vi "MouseDown.vi"(7 "Flip colors?":bool, 8 "error in":errorcluster, 10 "Coords":T5, 11 "Data in":T1={"Class"={"Ants"=refnum, "Layer"=refnum, "Templates"=refnum, "Icon"=refnum, "Glyph"=refnum, "Settings"=refnum, "Tools"=refnum, "History"=refnum}, "Ref"={"Add Layer"=refnum, "Remove Layer"=refnum, "Line Text"=[], "Body Text Spec"=refnum, "DNL_Font"=refnum, "glyph path str"=refnum, "templates path str"=refnum, "Arrow Up"=refnum, "Arrow Down"=refnum, "IE VI Ref"=refnum, "Glyphs tree"=refnum, "Templates tree"=refnum, "Layer Icon Text"=refnum, "Layer Template"=refnum, "Body Text"=refnum, "Search Templates"=refnum, "TextMarker"=refnum, "Tab Control"=refnum, "Search Glyphs"=refnum, "Line Color"=refnum, "DNL_Glyphs []"=refnum, "Fill Color"=refnum, "Tools"=refnum, "Icon"=refnum, "Preview"=refnum, "Ants"=refnum, "Terminals"=refnum, "menu reference"=refnum, "LayerNames"=[], "GlyphLoadAnimation"=refnum, "TemplateLoadAnimation"=refnum, "refreshGlyphs"=refnum, "refreshTemplates"=refnum}, "Support"={"AntsRect"={"left"=0, "top"=0, "right"=0, "bottom"=0}, "Mouse Move Coords"={"Horizontal"=0, "Vertical"=0}, "Mouse Down Coords"={"Horizontal"=0, "Vertical"=0}, "Temp Coord"={"Horizontal"=0, "Vertical"=0}, "Action"=enum."Default", "Edge Color"=4914962, "Fill Color"=16860, "Mouse Down?"=FALSE, "Draft Mode?"=FALSE, "Temp Icon"=bytes[3102], "CTRL Pressed"=FALSE, "Move Selection?"=FALSE, "AntsRect Orig"={"left"=0, "top"=0, "right"=0, "bottom"=0}, "Text"="", "TM Set?"=FALSE, "Mouse inside icon?"=FALSE, "Tool (old value)"=0, "Pencil Move Color"=0, "Swap Colors?"=FALSE, "Shift pressed?"=FALSE}}) -> (0 "error out":errorcluster, 3 "Data out":T1={"Class"={"Ants"=refnum, "Layer"=refnum, "Templates"=refnum, "Icon"=refnum, "Glyph"=refnum, "Settings"=refnum, "Tools"=refnum, "History"=refnum}, "Ref"={"Add Layer"=refnum, "Remove Layer"=refnum, "Line Text"=[], "Body Text Spec"=refnum, "DNL_Font"=refnum, "glyph path str"=refnum, "templates path str"=refnum, "Arrow Up"=refnum, "Arrow Down"=refnum, "IE VI Ref"=refnum, "Glyphs tree"=refnum, "Templates tree"=refnum, "Layer Icon Text"=refnum, "Layer Template"=refnum, "Body Text"=refnum, "Search Templates"=refnum, "TextMarker"=refnum, "Tab Control"=refnum, "Search Glyphs"=refnum, "Line Color"=refnum, "DNL_Glyphs []"=refnum, "Fill Color"=refnum, "Tools"=refnum, "Icon"=refnum, "Preview"=refnum, "Ants"=refnum, "Terminals"=refnum, "menu reference"=refnum, "LayerNames"=[], "GlyphLoadAnimation"=refnum, "TemplateLoadAnimation"=refnum, "refreshGlyphs"=refnum, "refreshTemplates"=refnum}, "Support"={"AntsRect"={"left"=0, "top"=0, "right"=0, "bottom"=0}, "Mouse Move Coords"={"Horizontal"=0, "Vertical"=0}, "Mouse Down Coords"={"Horizontal"=0, "Vertical"=0}, "Temp Coord"={"Horizontal"=0, "Vertical"=0}, "Action"=enum."Default", "Edge Color"=4914962, "Fill Color"=16860, "Mouse Down?"=FALSE, "Draft Mode?"=FALSE, "Temp Icon"=bytes[3102], "CTRL Pressed"=FALSE, "Move Selection?"=FALSE, "AntsRect Orig"={"left"=0, "top"=0, "right"=0, "bottom"=0}, "Text"="", "TM Set?"=FALSE, "Mouse inside icon?"=FALSE, "Tool (old value)"=0, "Pencil Move Color"=0, "Swap Colors?"=FALSE, "Shift pressed?"=FALSE}})   [LabVIEW 2020]
uses:
  Class/Ants/Ants.lvclass
  Class/FakedArray/FakedArray.lvclass
  vi.lib/LabVIEW Icon API/lv_icon/Classes/Icon/Icon.lvclass
  Class/Icon Library/Glyph.lvclass
  Class/Settings/Settings.lvclass
  Class/Tools/Tools Paint.lvclass
  History/History/History.lvclass
  Controls/SupportClass_Action.ctl
  History/History.lvlib
  <vilib>/Utility/miscctls.llb/LVPoint32TypeDef.ctl
  vi.lib/LabVIEW Icon API/lv_icon/Controls/IEColor.ctl
  Controls/Support Cluster.ctl
  lv_icon.lvlib
  Controls/References Cluster.ctl
  Controls/IE Classes.ctl
  Controls/Global Data.ctl
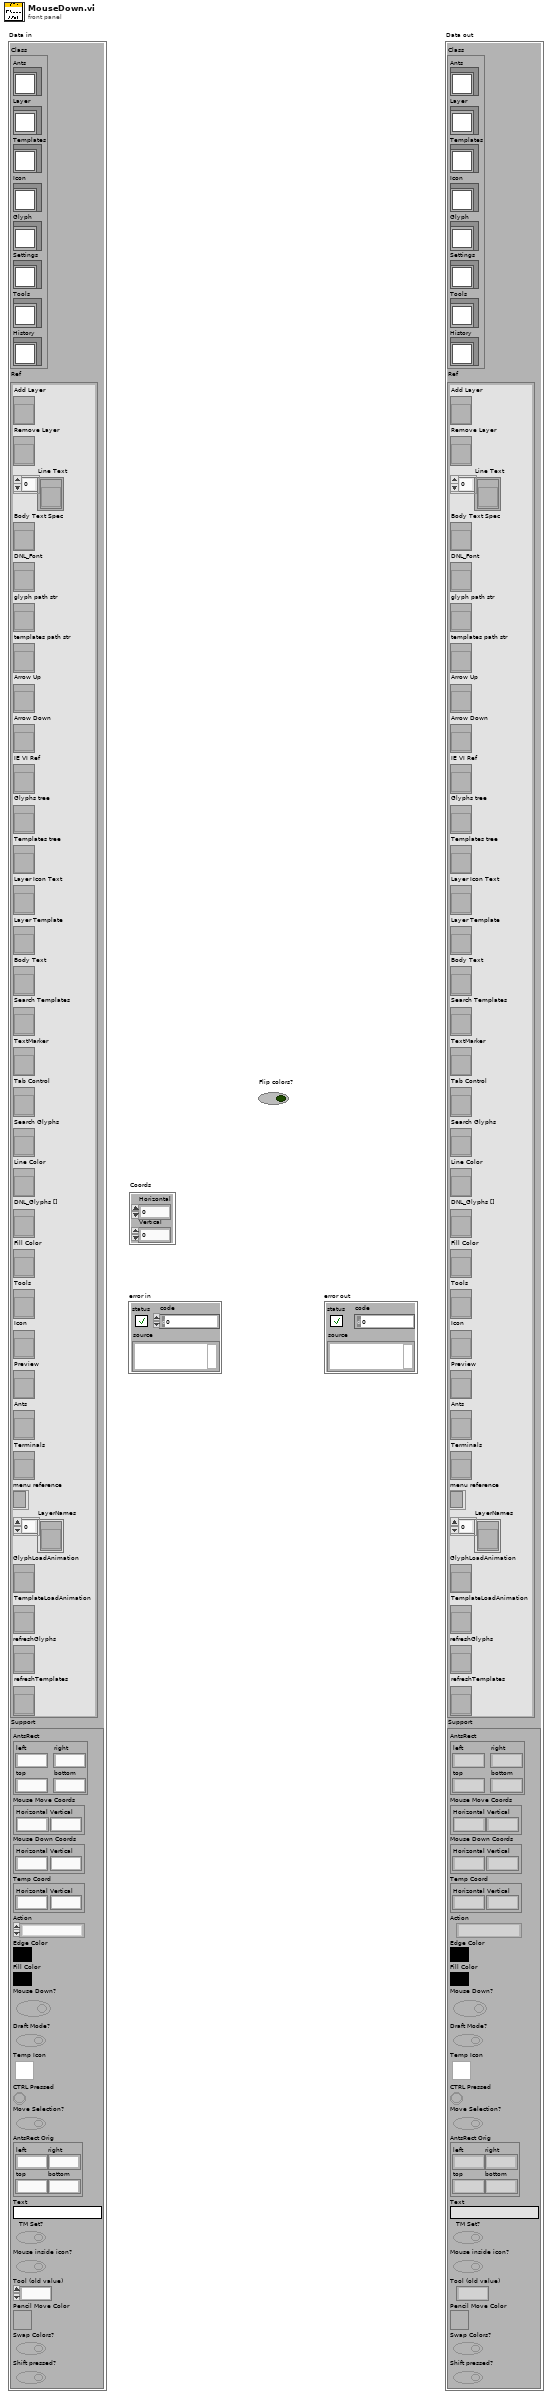
[diagram p1: front panel]
types:
  T1 = typedef "lv_icon.lvlib/Global Data.ctl" = cluster{"Class":T2, "Ref":T3, "Support":T4}
  T2 = typedef "lv_icon.lvlib/IE Classes.ctl" = cluster{"Ants":refnum<class "Ants.lvclass">, "Layer":refnum<class "FakedArray.lvclass">, "Templates":refnum<class "FakedArray.lvclass">, "Icon":refnum<class "Icon.lvclass">, "Glyph":refnum<class "Glyph.lvclass">, "Settings":refnum<class "Settings.lvclass">, "Tools":refnum<class "Tools Paint.lvclass">, "History":refnum<class "History.lvclass">}
  T3 = typedef "lv_icon.lvlib/References Cluster.ctl" = cluster{"Add Layer":refnum<vi>, "Remove Layer":refnum<vi>, "Line Text":refnum<vi>[], "Body Text Spec":refnum<vi>, "DNL_Font":refnum<vi>, "glyph path str":refnum<vi>, "templates path str":refnum<vi>, "Arrow Up":refnum<vi>, "Arrow Down":refnum<vi>, "IE VI Ref":refnum<vi>, "Glyphs tree":refnum<vi>, "Templates tree":refnum<vi>, "Layer Icon Text":refnum<vi>, "Layer Template":refnum<vi>, "Body Text":refnum<vi>, "Search Templates":refnum<vi>, "TextMarker":refnum<vi>, "Tab Control":refnum<vi>, "Search Glyphs":refnum<vi>, "Line Color":refnum<vi>, "DNL_Glyphs []":refnum<vi>, "Fill Color":refnum<vi>, "Tools":refnum<vi>, "Icon":refnum<vi>, "Preview":refnum<vi>, "Ants":refnum<vi>, "Terminals":refnum<vi>, "menu reference":refnum<k9>, "LayerNames":refnum<vi>[], "GlyphLoadAnimation":refnum<vi>, "TemplateLoadAnimation":refnum<vi>, "refreshGlyphs":refnum<vi>, "refreshTemplates":refnum<vi>}
  T4 = typedef "lv_icon.lvlib/Support Cluster.ctl" = cluster{"AntsRect":cluster{"left":i16, "top":i16, "right":i16, "bottom":i16}, "Mouse Move Coords":T5, "Mouse Down Coords":T5, "Temp Coord":T5, "Action":T6, "Edge Color":T7, "Fill Color":T7, "Mouse Down?":bool, "Draft Mode?":bool, "Temp Icon":picture, "CTRL Pressed":bool, "Move Selection?":bool, "AntsRect Orig":cluster{"left":i16, "top":i16, "right":i16, "bottom":i16}, "Text":string, "TM Set?":bool, "Mouse inside icon?":bool, "Tool (old value)":u32, "Pencil Move Color":u32, "Swap Colors?":bool, "Shift pressed?":bool}
  T5 = typedef "LVPoint32TypeDef.ctl" = cluster{"Horizontal":i32, "Vertical":i32}
  T6 = typedef "SupportClass_Action.ctl" = enum16{"Default", "Move Selection", "Glyph Library", "Tool"}
  T7 = typedef "IEColor.ctl" = u32
  T8 = cluster{"left":i16, "top":i16, "right":i16, "bottom":i16}
  T9 = typedef "Tools.ctl" = enum32{"Pencil", "Line", "Dropper", "Fill", "Rectangle", "Filled Rectangle", "Ellipse", "Filled Ellipse", "Eraser", "Text", "Select", "Move"}
  T10 = cluster{"Horizontal":i32, "Vertical":i32, "Vertical 2":i32, "Vertical 3":i32}
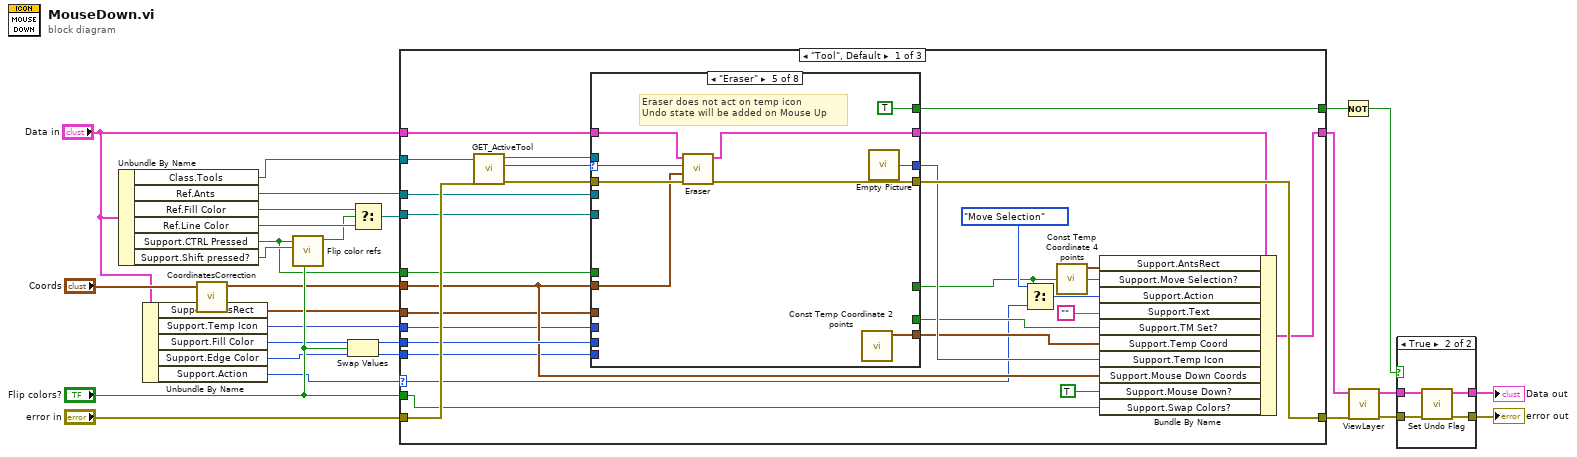
[diagram p0: block diagram]
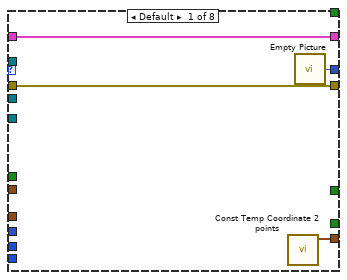
[diagram p3: hidden frame]
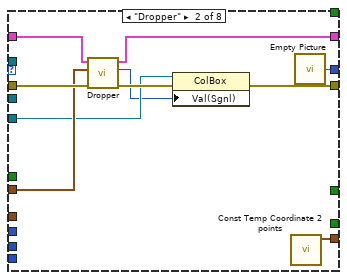
[diagram p4: hidden frame]
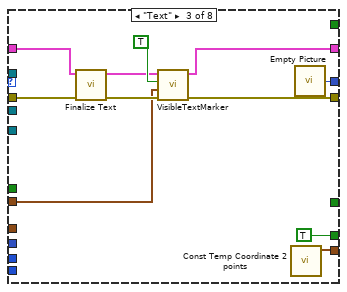
[diagram p5: hidden frame]
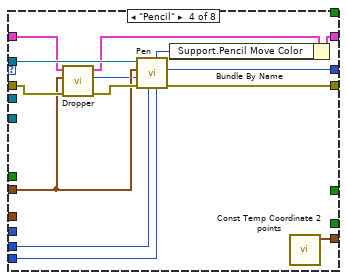
[diagram p6: hidden frame]
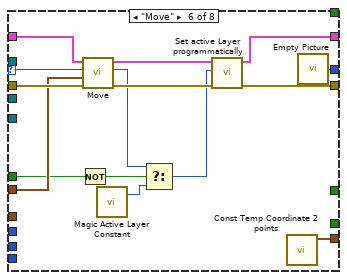
[diagram p7: hidden frame]
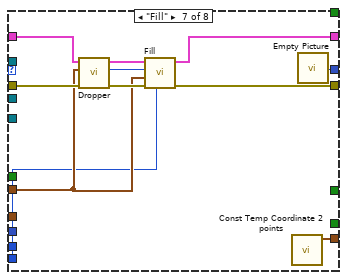
[diagram p8: hidden frame]
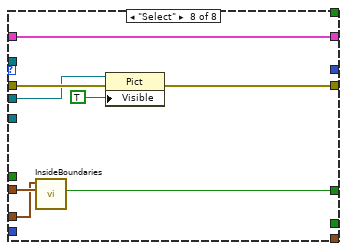
[diagram p9: hidden frame]
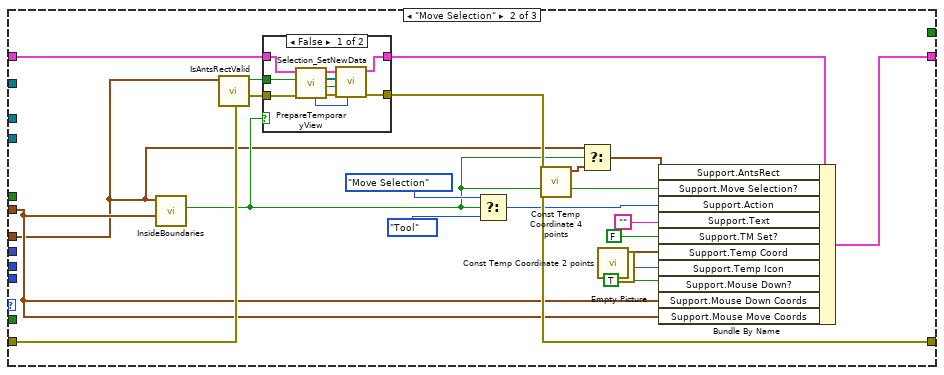
[diagram p10: hidden frame]
diagram:
  n1 = Unbundle By Name("Data in") -> ("Class.Tools"=w17:refnum<class "Tools Paint.lvclass">, "Ref.Ants"=w19:refnum<vi>, "Ref.Fill Color"=w9:refnum<vi>, "Ref.Line Color"=w8:refnum<vi>, "Support.CTRL Pressed"=w5:bool, "Support.Shift pressed?"=w6:bool)
  n2 = Unbundle By Name("Data in") -> ("Support.AntsRect"=w18:T8, "Support.Temp Icon"=w20:picture, "Support.Fill Color"=w12:T7, "Support.Edge Color"=w14:T7, "Support.Action"=w22:T6)
  n3 = call "CoordinatesCorrection.vi"("Coordinates In"="Coords") -> ("Corrected Out"=w23:T5)  [unwired: 10 out]
  n4 = call "Flip color refs.vi"("Flip colors?"="Flip colors?", "Shift pressed"=w6, "CTRL pressed"=w5) -> ("Flip?"=w7:bool)  [unwired: 8 out]
  n5 = Swap Values(12:w12, 13:"Flip colors?", 14:w14) -> (1:w11:T7, 3:w13:T7)
  n6 = Select(t=w9, s=w7, f=w8) -> (s? t:f=w10:refnum<vi>)
  n7 = case shown="\"Tool\", Default" w22 {
    selector: w22 -> [w41 _ _]
    tunnel: [w56 w157 w172] -> w26
    tunnel: w23 -> [w51 w147 _]
    tunnel: "error in" -> [w55 w158 w172]
    tunnel: [w49 w152 w171] -> w15
    tunnel: w11 -> [w52 _ _]
    tunnel: w13 -> [w48 _ _]
    tunnel: w20 -> [w45 _ _]
    tunnel: w19 -> [w44 _ _]
    tunnel: w18 -> [w43 w142 _]
    tunnel: w10 -> [w37 _ _]
    tunnel: w17 -> [w35 _ _]
    tunnel: "Data in" -> [w34 w145 w171]
    tunnel: "Flip colors?" -> [w33 _ _]
    tunnel: w5 -> [w31 _ _]
    tunnel: [w29 _ _] -> w2
    frame "Tool", Default {
      n8 = call-dynamic "GET_ActiveTool.vi"("error in (no error)"=w55, "Tools Paint.lvclass in"=w35) -> ("error out"=w57:errorcluster, "Radio Buttons"=w54:T9, "Tools Paint.lvclass out"=w38:refnum<class "Tools Paint.lvclass">)  [unwired: 7 out]
      n9 = case shown="\"Eraser\"" w54 {
        selector: w54 -> [_ _ _ _ w101 w115 _ _]
        tunnel: w57 -> [w61 w71 w81 w95 w105 w120 w129 w138]
        tunnel: w51 -> [_ w67 w72 w90 w102 w116 w126 w135]
        tunnel: w52 -> [_ _ _ w83 _ _ _ _]
        tunnel: [w60 w68 w77 w93 w103 w117 w127 _] -> w50
        tunnel: [w61 w70 w82 w96 w104 w118 w131 w139] -> w56
        tunnel: w48 -> [_ _ _ w84 _ _ w121 _]
        tunnel: [w59 w66 w79 w92 w100 w114 w128 _] -> w47
        tunnel: [_ _ TRUE ("Mouse Down?") _ _ _ _ _] -> w46
        tunnel: w45 -> [_ _ _ _ _ _ _ _]
        tunnel: w44 -> [_ _ _ _ _ _ _ w137]
        tunnel: w43 -> [_ _ _ _ _ _ _ w134]
        tunnel: [_ _ _ _ _ _ _ w133] -> w36
        tunnel: w38 -> [_ _ _ w91 _ _ _ _]
        tunnel: w37 -> [_ w65 _ _ _ _ _ _]
        tunnel: w34 -> [w58 w64 w76 w88 w99 w113 w124 w132]
        tunnel: [w58 w63 w73 w86 w98 w111 w122 w132] -> w30
        tunnel: w31 -> [_ _ _ _ _ w110 _ _]
        tunnel: [_ _ _ _ TRUE _ _ _] -> w29
        frame Default {
          n10 = call "Const Temp Coordinate 2 points.vi"() -> ("Const Temp Coordinate"=w59:T5)  [unwired: 11 out]
          n11 = call "Empty Picture"() -> ("empty picture"=w60:picture)
        }
        frame "Dropper" {
          n12 = call "Dropper.vi"("error in (no error)"=w71, "point(x,y)"=w67, "Data in"=w64) -> ("error out"=w69:errorcluster, "Color"=w62:u32, "Data out"=w63:T1)  [unwired: 1 in, 5 out]
          n13 = property on="Property Node" class="ColBox"(reference=w65, error in=w69, "Val(Sgnl)"=w62) -> (error out=w70:errorcluster)  [unwired: 1 out]
          n14 = call "Const Temp Coordinate 2 points.vi"() -> ("Const Temp Coordinate"=w66:T5)  [unwired: 11 out]
          n15 = call "Empty Picture"() -> ("empty picture"=w68:picture)
        }
        frame "Text" {
          n16 = call "Finalize Text.vi"("error in (no error)"=w81, "Data in"=w76) -> ("error out"=w80:errorcluster, "Data out"=w74:T1)  [unwired: 8 out]
          n17 = call "VisibleTextMarker.vi"("error in"=w80, "Position"=w72, "Visible"=TRUE, "Data in"=w74) -> ("error out"=w82:errorcluster, "Data out"=w73:T1)  [unwired: 6 out]
          n18 = call "Const Temp Coordinate 2 points.vi"() -> ("Const Temp Coordinate"=w79:T5)  [unwired: 11 out]
          n19 = call "Empty Picture"() -> ("empty picture"=w77:picture)
        }
        frame "Pencil" {
          n20 = call "Dropper.vi"("error in (no error)"=w95, "point(x,y)"=w90, "Data in"=w88) -> ("error out"=w94:errorcluster, "Color"=w89:u32, "Data out"=w87:T1)  [unwired: 6 out]
          n21 = call-dynamic "Pen.vi"("Edge color"=w84, "Fill color"=w83, "error in (no error)"=w94, "Current color (T)"=w89, "point(x,y)"=w90, "Tools Paint in"=w91) -> ("error out"=w96:errorcluster, "new picture"=w93:picture, "Current line color"=w85:u32)  [unwired: 3 out]
          n22 = Bundle By Name(cluster=w87, "Support.Pencil Move Color"=w85) -> (w86:T1)
          n23 = call "Const Temp Coordinate 2 points.vi"() -> ("Const Temp Coordinate"=w92:T5)  [unwired: 11 out]
        }
        frame "Eraser" {
          # "Eraser does not act on temp icon\nUndo state will be added on Mouse Up"
          n24 = call "Eraser.vi"("error in (no error)"=w105, "point(x,y)"=w102, "Radio Buttons"=w101, "Data in"=w99) -> ("error out"=w104:errorcluster, "Data out"=w98:T1)  [unwired: 1 in, 5 out]
          n25 = call "Const Temp Coordinate 2 points.vi"() -> ("Const Temp Coordinate"=w100:T5)  [unwired: 11 out]
          n26 = call "Empty Picture"() -> ("empty picture"=w103:picture)
        }
        frame "Move" {
          n27 = Not(x=w110) -> (.not. x?=w109:bool)
          n28 = call "Move.vi"("error in (no error)"=w120, "point(x,y)"=w116, "Tools"=w115, "Data in"=w113) -> ("error out"=w119:errorcluster, "Active Layer"=w108:i32, "Data out"=w112:T1)  [unwired: 1 in, 4 out]
          n29 = call "Magic Active Layer Constant.vi"() -> ("Magic Constant"=w107:i32)  [unwired: 19 out]
          n30 = Select(t=w108, s=w109, f=w107) -> (s? t:f=w106:i32)
          n31 = call "Set active Layer programmatically.vi"("error in"=w119, "Active Layer"=w106, "Data in"=w112) -> ("error out"=w118:errorcluster, "Data out"=w111:T1)  [unwired: 1 in, 6 out]
          n32 = call "Const Temp Coordinate 2 points.vi"() -> ("Const Temp Coordinate"=w114:T5)  [unwired: 11 out]
          n33 = call "Empty Picture"() -> ("empty picture"=w117:picture)
        }
        frame "Fill" {
          n34 = call "Dropper.vi"("error in (no error)"=w129, "point(x,y)"=w126, "Data in"=w124) -> ("error out"=w130:errorcluster, "Color"=w125:u32, "Data out"=w123:T1)  [unwired: 6 out]
          n35 = call "Fill.vi"("Color"=w121, "error in (no error)"=w130, "point(x,y)"=w126, "Ref Color"=w125, "Data in"=w123) -> ("error out"=w131:errorcluster, "Data out"=w122:T1)  [unwired: 1 in, 4 out]
          n36 = call "Const Temp Coordinate 2 points.vi"() -> ("Const Temp Coordinate"=w128:T5)  [unwired: 11 out]
          n37 = call "Empty Picture"() -> ("empty picture"=w127:picture)
        }
        frame "Select" {
          n38 = call "InsideBoundaries.vi"("Mouse Move Coords"=w135, "AntsRect"=w134) -> ("Inside?"=w133:bool)  [unwired: 9 out]
          n39 = property class="Pict"(reference=w137, error in=w138, "Visible"=TRUE) -> (error out=w139:errorcluster)  [unwired: 1 out]
        }
      }
      n40 = Select(t=SupportClass_Action."Move Selection", s=w36, f=w41) -> (s? t:f=w39:T6)
      n41 = call "Const Temp Coordinate 4 points.vi"() -> ("Const Temp Coordinate"=w32:T10)  [unwired: 11 out]
      n42 = Bundle By Name(cluster=w30, "Support.AntsRect"=w32, "Support.Move Selection?"=w36, "Support.Action"=w39, "Support.Text"="", "Support.TM Set?"=w46, "Support.Temp Coord"=w47, "Support.Temp Icon"=w50, "Support.Mouse Down Coords"=w51, "Support.Mouse Down?"=TRUE ("Mouse Down?"), "Support.Swap Colors?"=w33) -> (w49:T1)
    }
    frame "Move Selection" {
      n43 = call "InsideBoundaries.vi"("Mouse Move Coords"=w147, "AntsRect"=w142) -> ("Inside?"=w143:bool)  [unwired: 9 out]
      n44 = call "IsAntsRectValid.vi"("AntsRect"=w142) -> ("Valid?"=w146:bool)  [unwired: 10 out]
      n45 = case shown="False" w143 {
        tunnel: w146 -> [w162 _]
        tunnel: w158 -> [w168 w170]
        tunnel: [w167 w170] -> w157
        tunnel: w145 -> [w161 w169]
        tunnel: [w159 w169] -> w144
        frame False {
          n46 = call "PrepareTemporaryView.vi"("error in (no error)"=w168, "Valid Selection?"=w162, "Data in"=w161) -> ("error out"=w166:errorcluster, "Highlighted?"=w164:bool, "All Layers out"=w165:refnum<class "Layer.lvclass">[], "Data out"=w160:T1, "#Active Layer"=w163:i32)  [unwired: 2 in, 2 out]
          n47 = call "Selection_SetNewData.vi"("#Active Layer"=w163, "error in"=w166, "Highlighted?"=w164, "All Layers In"=w165, "Data in"=w160) -> ("error out"=w167:errorcluster, "Data out"=w159:T1)  [unwired: 1 in, 3 out]
        }
        frame True {
        }
      }
      n48 = Select(t=SupportClass_Action."Move Selection", s=w143, f=SupportClass_Action."Tool") -> (s? t:f=w151:T6)
      n49 = call "Const Temp Coordinate 4 points.vi"() -> ("Const Temp Coordinate"=w141:T10)  [unwired: 11 out]
      n50 = Select(t=w142, s=w143, f=w141) -> (s? t:f=w140:T10)
      n51 = call "Const Temp Coordinate 2 points.vi"() -> ("Const Temp Coordinate"=w150:T5)  [unwired: 11 out]
      n52 = call "Empty Picture"() -> ("empty picture"=w149:picture)
      n53 = Bundle By Name(cluster=w144, "Support.AntsRect"=w140, "Support.Move Selection?"=w143, "Support.Action"=w151, "Support.Text"="", "Support.TM Set?"=FALSE ("TM Set?"), "Support.Temp Coord"=w150, "Support.Temp Icon"=w149, "Support.Mouse Down?"=TRUE ("Mouse Down?"), "Support.Mouse Down Coords"=w147, "Support.Mouse Move Coords"=w147) -> (w152:T1)
    }
    frame "Glyph Library" {
    }
  }
  n54 = Not(x=w2) -> (.not. x?=w1:bool)
  n55 = call "ViewLayer.vi"("error in (no error)"=w26, "Data in"=w15) -> ("error out"=w25:errorcluster, "Data out"=w4:T1)  [unwired: 2 in, 6 out]
  n56 = case shown="True" w1 {
    tunnel: w25 -> [w174 w178]
    tunnel: [w174 w177] -> w24
    tunnel: w4 -> [w173 w176]
    tunnel: [w173 w175] -> w3
    frame False {
    }
    frame True {
      n57 = call "Set Undo Flag.vi"("error in"=w178, "Data in"=w176) -> ("error out"=w177:errorcluster, "Data out"=w175:T1)  [unwired: 8 in]
    }
  }
  "error out" <- w24
  "Data out" <- w3
